vi "Test MQTT-3.1.3-9.vi"(8 "error in (no error)":errorcluster, 11 "Connection Config":refnum<class "Connection.lvclass">) -> (0 "error out":errorcluster, 3 "Connection Config dup":refnum<class "Connection.lvclass">)   [LabVIEW 2013]
uses:
  <vilib>/LabVIEW Open Source Project/MQTT Control Packets/Control Packets/CONNECT/CONNECT.lvclass
  <vilib>/LabVIEW Open Source Project/MQTT Control Packets/Control Packets/ControlPacket/ControlPacket.lvclass
  <vilib>/addons/_JKI Toolkits/Caraya/classes/Test/Test.lvclass
  <vilib>/LabVIEW Open Source Project/MQTT Control Packets/Control Packets/DISCONNECT/DISCONNECT.lvclass
  <vilib>/LabVIEW Open Source Project/MQTT Control Packets/Control Packets/CONNACK/CONNACK.lvclass
  <vilib>/LabVIEW Open Source Project/MQTT Control Packets/Control Packets/CONNACK/Connect Return Code -- enum.ctl
  <vilib>/addons/_JKI Toolkits/Caraya/classes/Assert/Assert.lvclass
  <vilib>/LabVIEW Open Source Project/Connection/Connection/Connection.lvclass
  <vilib>/LabVIEW Open Source Project/MQTT Connection/MQTT_Connection/Connection/Connection.lvclass
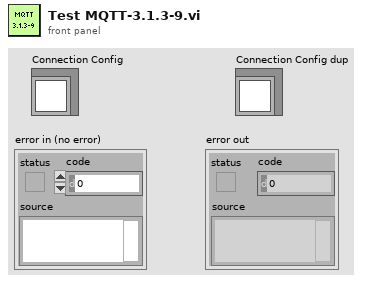
[diagram p1: front panel]
types:
  T1 = typedef "MQTT_Control_Packets.lvlib/CONNACK.lvclass/Connect Return Code -- enum.ctl" = enum16{"Connection accepted", "Unacceptable protocol version", "Identifier Rejected", "Server Unavailable", "Bad Username or Password", "Not Authorized"}
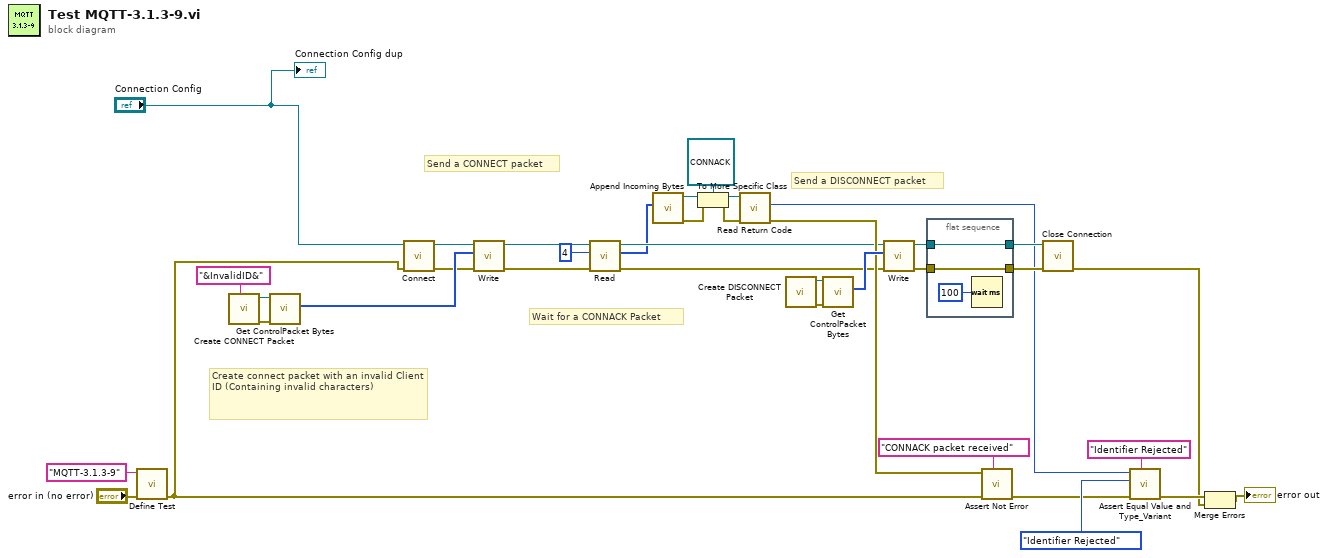
[diagram p0: block diagram]
diagram:
  # "Send a DISCONNECT packet"
  # "Wait for a CONNACK Packet"
  # "Create connect packet with an invalid Client ID (Containing invalid characters)"
  # "Send a CONNECT packet"
  n1 = call <vilib>:"Define Test.vi"("error in (no error)"="error in (no error)", "Label (VI Title)"="MQTT-3.1.3-9") -> ("error out"=w1:errorcluster)  [unwired: 9 in]
  n2 = call <vilib>:"Create CONNECT Packet.vi"("Client ID (empty: generate new)"="&InvalidID&") -> ("error out"=w36:errorcluster, "CONNECT"=w37:refnum<class "CONNECT.lvclass">)  [unwired: 8 in, 1 out]
  n3 = call <vilib>:"Get ControlPacket Bytes.vi"("error in (no error)"=w36, "ControlPacket"=w37) -> ("Bytes Stream"=w7:u8[])  [unwired: 6 in, 3 out]
  n4 = call <vilib>:"Connect.vi"("error in (no error)"=w1, "Connection in"="Connection Config") -> ("error out"=w5:errorcluster, "Connection out"=w6:refnum<class "Connection.lvclass">)  [unwired: 8 in]
  n5 = call <vilib>:"Write.vi"("error in (no error)"=w5, "Bytes"=w7, "Connection in"=w6) -> ("error out"=w12:errorcluster, "Connection"=w13:refnum<class "Connection.lvclass">)  [unwired: 7 in]
  n6 = call <vilib>:"Read.vi"("error in (no error)"=w12, "bytes to read (100)"=4 ("bytes to read"), "TCPConnection in"=w13) -> ("error out"=w10:errorcluster, "Bytes"=w9:u8[], "TCPConnection out"=w11:refnum<class "Connection.lvclass">)  [unwired: 4 in, 2 out]
  n7 = call <vilib>:"Append Incoming Bytes.vi"("Incoming Packets"=w9) -> ("error out"=w15:errorcluster, "ControlPacket"=w23:refnum<class "ControlPacket.lvclass">)  [unwired: 7 in, 2 out]
  n8 = To More Specific Class(target class=refnum<class "CONNACK.lvclass"> refnum ("CONNACK in"), reference=w23, error in=w15) -> (specific class reference=w22:refnum<class "CONNACK.lvclass">, error out=w19:errorcluster)
  n9 = call <vilib>:"Read Return Code.vi"("error in (no error)"=w19, "CONNACK in"=w22) -> ("error out"=w17:errorcluster, "Return Code"=w4:T1)  [unwired: 7 in, 1 out]
  n10 = call <vilib>:"Create DISCONNECT Packet.vi"() -> ("error out"=w29:errorcluster, "DISCONNECT"=w28:refnum<class "DISCONNECT.lvclass">)  [unwired: 9 in, 1 out]
  n11 = call <vilib>:"Get ControlPacket Bytes.vi"("error in (no error)"=w29, "ControlPacket"=w28) -> ("Bytes Stream"=w27:u8[])  [unwired: 6 in, 3 out]
  n12 = call <vilib>:"Write.vi"("error in (no error)"=w10, "Bytes"=w27, "Connection in"=w11) -> ("error out"=w25:errorcluster, "Connection"=w26:refnum<class "Connection.lvclass">)  [unwired: 7 in]
  n13 = flat-sequence {
    tunnel: w26 -> [w40]
    tunnel: [w40] -> w24
    tunnel: [w38] -> w21
    tunnel: w25 -> [w38]
    frame #0 {
      n14 = Wait (ms)(milliseconds to wait=u32 100) -> ()  [unwired: 1 out]
    }
  }
  n15 = call <vilib>:"Assert Not Error.vi"("Label"="CONNACK packet received", "error in (no error)"=w1, "Not Error?"=w17) -> ("error out"=w18:errorcluster)  [unwired: 8 in]
  n16 = call <vilib>:"Close Connection.vi"("error in (no error)"=w21, "Connection in"=w24) -> ("error out"=w31:errorcluster)  [unwired: 8 in, 1 out]
  n17 = call <vilib>:"Assert Equal Value and Type_Variant.vi"("Label"="Identifier Rejected", "error in (no error)"=w18, "Y"=Connect_Return_Code_--_enum."Identifier Rejected" ("Return Code"), "X"=w4) -> ("error out"=w34:errorcluster)  [unwired: 7 in]
  n18 = Merge Errors(w34, w31) -> (→"error out":errorcluster)
  "Connection Config dup" <- "Connection Config"
